vi "Shutdown.vi"(7 "FPGA ref":refnum<k20>, 8 "error in (no error)":errorcluster, 10 "rt fifo ref in":refnum<k33>, 11 "cdm reader":refnum<k21>) -> (0 "error out":errorcluster)   [LabVIEW 2025]
uses:
  RT_Cmd.ctl
  Command.ctl
  vi/thresholds.ctl
  <vilib>/rvi/interface/nirviCloseFPGA/nirviCloseFPGA.xnode
  <vilib>/FPGAPlugInAG/Dynamic/niLvFpga_Close_Dynamic.vi
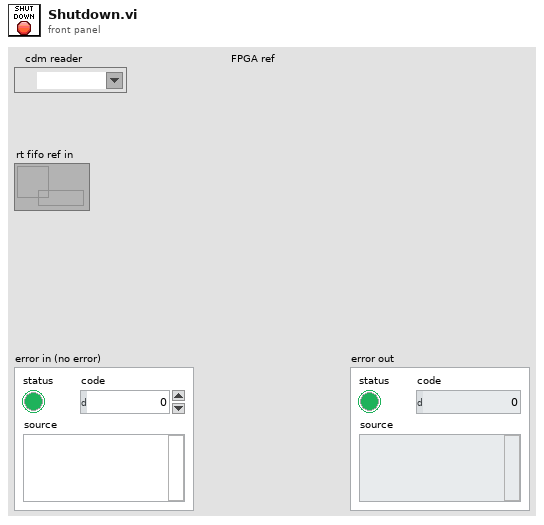
[diagram p1: front panel]
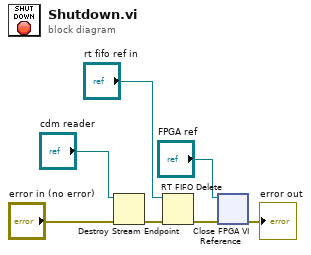
[diagram p0: block diagram]
diagram:
  n1 = Destroy Stream Endpoint(8:"error in (no error)", 11:"cdm reader") -> (0:w6:errorcluster)
  n2 = RT FIFO Delete(0:"rt fifo ref in", 3:w6) -> (11:w3:errorcluster)  [unwired: 1 in]
  n3 = xnode "Close FPGA VI Reference"("FPGA VI Reference In"="FPGA ref", "error in"=w3) -> ("error out"=→"error out":errorcluster)
